vi "Read Volatus INI.vi"(8 "error in (no error)":errorcluster, 10 "INI Path (Default)":path, 11 "Volatus Core in":refnum<class "Volatus Core.lvclass">) -> (0 "error out":errorcluster, 3 "Volatus Core out":refnum<class "Volatus Core.lvclass">)   [LabVIEW 2020, in "Volatus.lvlib" / "Volatus Core.lvclass"]
uses:
  Volatus Core.lvclass
  Volatus Core.lvclass/Volatus Core.ctl
  Volatus.lvlib
  <vilib>/Utility/config.llb/NI_LVConfig.lvlib
  <vilib>/Utility/config.llb/Read Key (String).vi
  Config Type.ctl
  lv-vecto/Vecto/Node Config/Node Info.ctl
  lv-vecto/VectoConfig/VectoConfig.lvlib
  lv-vecto/Vecto/Node Config/Node Config.lvclass
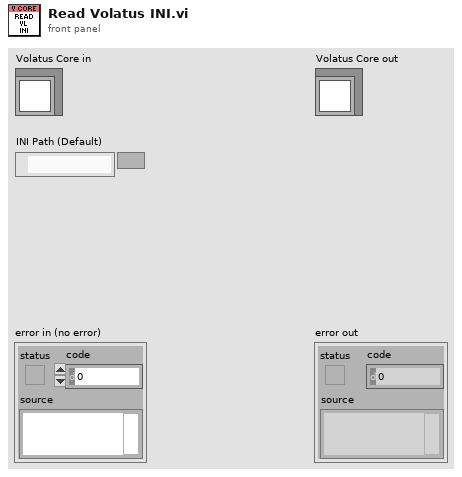
[diagram p1: front panel]
types:
  T1 = typedef "Volatus.lvlib/Volatus Core.lvclass/Config Type.ctl" = enum16{"App INI", "Memory", "Unconfigured"}
  T2 = typedef "VectoConfig.lvlib/Node Info.ctl" = cluster{"System":string, "Cluster":string, "Name":string, "ID":u32, "Capabilities":string[]}
  T3 = typedef "NI_LVConfig.lvlib/Config Data RefNum.ctl" = refnum<k1>
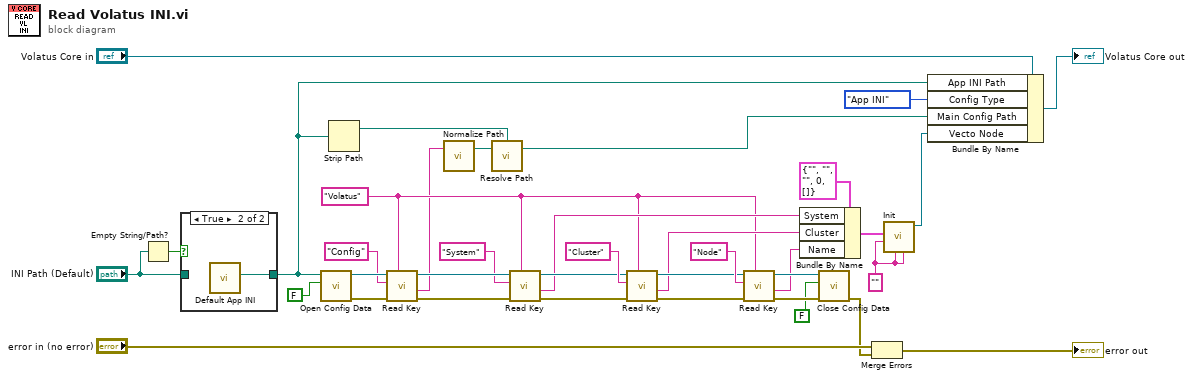
[diagram p0: block diagram]
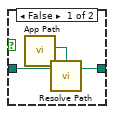
[diagram p2: hidden frame]
diagram:
  w1 = "" ("Config Version")
  w10 = "Volatus" ("section")
  n1 = Empty String/Path?(string/path="INI Path (Default)") -> (empty?=w9:bool)
  n2 = case shown="True" w9 {
    tunnel: [w39 w41] -> w2
    tunnel: "INI Path (Default)" -> [w40 _]
    frame False {
      n3 = call "App Path.vi"() -> ("App Path"=w38:path)  [unwired: 11 in]
      n4 = call "Resolve Path.vi"("Starting Path"=w38, "Path"=w40) -> ("Resolved Path"=w39:path)  [unwired: 4 in]
    }
    frame True {
      n5 = call "Default App INI.vi"() -> ("Default App INI"=w41:path)  [unwired: 11 in]
    }
  }
  n6 = call <vilib>:"Open Config Data.vi"("create file if necessary (T)"=FALSE, "configuration file path"=w2) -> ("error out"=w35:errorcluster, "refnum"=w34:T3)  [unwired: 7 in, 1 out]
  n7 = Strip Path(path=w2) -> (stripped path=w4:path)  [unwired: 1 out]
  n8 = call-poly <vilib>:"Read Key.vi"("section"=w10, "error in (no error)"=w35, "key"="Config" ("section"), "refnum"=w34) -> ("error out"=w30:errorcluster, "value"=w7:string, "refnum out"=w31:T3)  [unwired: 4 in, 1 out]
  n9 = call "Normalize Path.vi"("Path String"=w7) -> ("Path"=w5:path)  [unwired: 2 in]
  n10 = call "Resolve Path.vi"("Starting Path"=w4, "Path"=w5) -> ("Resolved Path"=w3:path)  [unwired: 4 in]
  n11 = call-poly <vilib>:"Read Key.vi"("section"=w10, "error in (no error)"=w30, "key"="System" ("section"), "refnum"=w31) -> ("error out"=w29:errorcluster, "value"=w18:string, "refnum out"=w28:T3)  [unwired: 4 in, 1 out]
  n12 = call-poly <vilib>:"Read Key.vi"("section"=w10, "error in (no error)"=w29, "key"="Cluster" ("section"), "refnum"=w28) -> ("error out"=w24:errorcluster, "value"=w17:string, "refnum out"=w25:T3)  [unwired: 4 in, 1 out]
  n13 = call-poly <vilib>:"Read Key.vi"("section"=w10, "error in (no error)"=w24, "key"="Node" ("section"), "refnum"=w25) -> ("error out"=w22:errorcluster, "value"=w16:string, "refnum out"=w23:T3)  [unwired: 4 in, 1 out]
  n14 = Bundle By Name(cluster=T2 {"System"="", "Cluster"="", "Name"="", "ID"=0, "Capabilities"=[]} ("Node Info"), "System"=w18, "Cluster"=w17, "Name"=w16) -> (w14:T2)
  n15 = call <vilib>:"Close Config Data.vi"("error in (no error)"=w22, "write file if changed (T)"=FALSE, "refnum"=w23) -> ("error out"=w19:errorcluster)  [unwired: 7 in, 1 out]
  n16 = Merge Errors("error in (no error)", w19) -> (→"error out":errorcluster)
  n17 = call "Init.vi"("Config Hash"=w1, "Config Version"=w1, "Alias (None)"=w1, "Node Info"=w14) -> ("Node out"=w13:refnum<class "Node Config.lvclass">)  [unwired: 6 in, 1 out]
  n18 = Bundle By Name(cluster="Volatus Core in", "App INI Path"=w2, "Config Type"=Config_Type."App INI", "Main Config Path"=w3, "Vecto Node"=w13) -> (→"Volatus Core out":refnum<class "Volatus Core.lvclass">)
